vi "lvmcp_propwrite.vi"() -> ()   [LabVIEW 2015]
panel:
  out "error out":errorcluster
  in  "write":bool
  in  "item":refnum<vi>
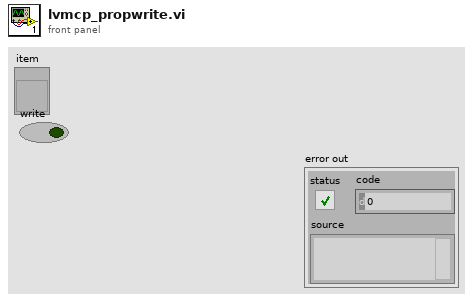
[diagram p1: front panel]
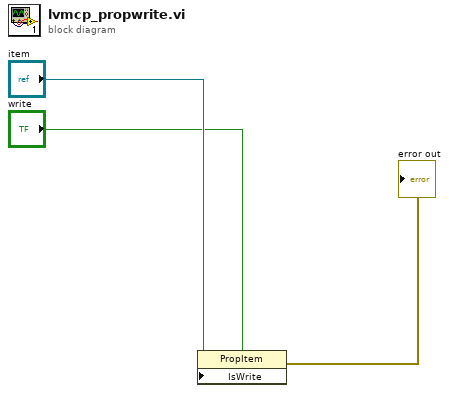
[diagram p0: block diagram]
diagram:
  n1 = property class="PropItem"(reference="item", "IsWrite"="write") -> (error out=→"error out":errorcluster)  [unwired: 1 in, 1 out]
